vi "VIH ProjFile - Control Rules Array - Read.vi"(8 "error in":errorcluster, 10 "Property Name":string, 11 "XML Parent Item":refnum<k20>) -> (0 "error out":errorcluster, 1 "Control Rules":T1[](array[typedef]), 2 "Property found":bool, 3 "dup XML Parent Item":refnum<k20>)   [LabVIEW 2014]
doc: "::: VI Helpeks :::\nCopyright (c) 2000-2026 Konstantin Shifershteyn. All rights reserved."
uses:
  _VIH HelpGen.llb/VIH HelpGen Typedef - Cluster - Control Rule.ctl
  _VIH HelpGen.llb/VIH HelpGen Typedef - Enum - Description Mode.ctl
  _VIH HelpGen.llb/VIH HelpGen Typedef - Enum - Default,Enable,Disable.ctl
  _VIH HelpGen.llb/VIH HelpGen Typedef - Cluster - Enum Value Info.ctl
  <vilib>/xml/Close Reference(Node).vi
  <vilib>/xml/NI_XML.lvlib
panel:
  in  "Control Rule (data)":T1
  # "VI Helpeks\nCopyright (c) 2012-2026 Konstantin Shifershteyn"
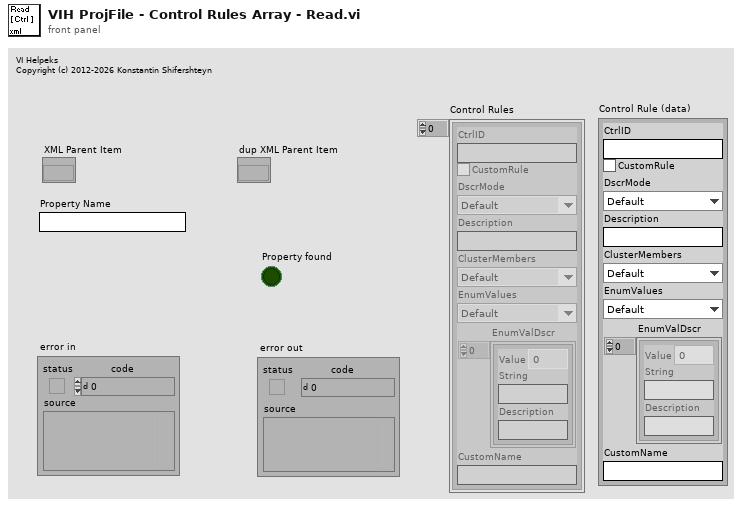
[diagram p1: front panel]
types:
  T1 = typedef "VIH HelpGen Typedef - Cluster - Control Rule.ctl" = cluster{"CtrlID":string, "CustomRule":bool, "DscrMode":T2, "Description":string, "ClusterMembers":T3, "EnumValues":T3, "EnumValDscr":T4[], "CustomName":string}
  T2 = typedef "VIH HelpGen Typedef - Enum - Description Mode.ctl" = enum16{"Default", "Description", "Description1", "Description2", "Custom", "None"}
  T3 = typedef "VIH HelpGen Typedef - Enum - Default,Enable,Disable.ctl" = enum16{"Default", "Enable", "Disable"}
  T4 = typedef "VIH HelpGen Typedef - Cluster - Enum Value Info.ctl" = cluster{"Value":ext, "String":string, "Description":string}
  T5 = typedef "KS HelpGen Typedef - Cluster - Control Rule.ctl" = cluster{"CtrlID":string, "CustomRule":bool, "DscrMode":T6, "Description":string, "ClusterMembers":T7, "EnumValues":T7, "EnumValDscr":T8[], "CustomName":string}
  T6 = typedef "KS HelpGen Typedef - Enum - Description Mode.ctl" = enum16{"Default", "Description", "Description1", "Description2", "Custom", "None"}
  T7 = typedef "KS HelpGen Typedef - Enum - Default,Enable,Disable.ctl" = enum16{"Default", "Enable", "Disable"}
  T8 = typedef "KS HelpGen Typedef - Cluster - Enum Value Info.ctl" = cluster{"Value":ext, "String":string, "Description":string}
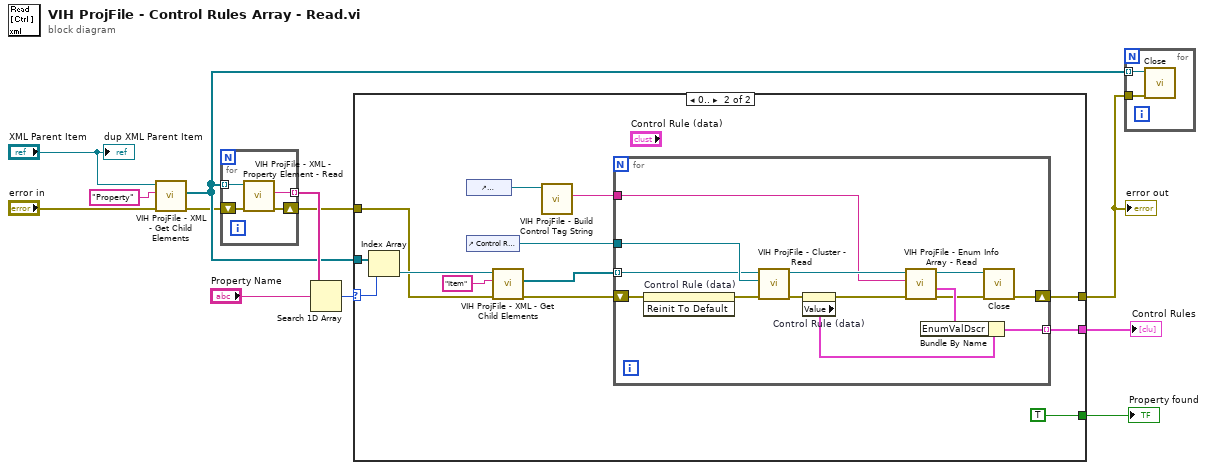
[diagram p0: block diagram]
diagram:
  n1 = call "VIH ProjFile - XML - Get Child Elements.vi"("error in"="error in", "Tag Name"="Property", "XML Parent Item"="XML Parent Item") -> ("error out"=w4:errorcluster, "Array of Elements"=w6:refnum<k20>[])  [unwired: 6 in, 1 out]
  n2 = for {
    tunnel: w6 -> [w16] mode=indexing
    shift-right: [w14] -> w10
    shift-left: w4 -> [w15]
    tunnel: [w13] -> w12 mode=indexing
    n3 = call "VIH ProjFile - XML - Property Element - Read.vi"("error in"=w15, "XML Node"=w16) -> ("error out"=w14:errorcluster, "Property Name"=w13:string)  [unwired: 6 in, 2 out]
  }
  n4 = Search 1D Array(1D array=w12, element="Property Name") -> (index of element=w11:i32)  [unwired: 1 in]
  n5 = case shown="0.." w11 {
    selector: w11 -> [_ w29]
    tunnel: [w17 w28] -> w8
    tunnel: w10 -> [w17 w22]
    tunnel: w6 -> [_ w30]
    tunnel: [_ w27] -> w9
    tunnel: [_ TRUE] -> w1
    frame ..-1 {
    }
    frame 0.. {
      n6 = Index Array(array=w30, index=w29) -> (element=w23:refnum<k20>)
      n7 = control-ref of="EnumValDscr"() -> (w26:refnum<vi>)
      n8 = control-ref of="Control Rule (data)"() -> (w25:refnum<vi>)
      n9 = call "VIH ProjFile - XML - Get Child Elements.vi"("error in"=w22, "Tag Name"="Item", "XML Parent Item"=w23) -> ("error out"=w20:errorcluster, "Array of Elements"=w21:refnum<k20>[])  [unwired: 6 in, 1 out]
      n10 = call "VIH ProjFile - Build Control Tag String.vi"("Ctl Refnum"=w26) -> ("Control Tag"=w24:string)  [unwired: 6 in, 4 out]
      n11 = for {
        tunnel: w21 -> [w31] mode=indexing
        shift-right: [w32] -> w28
        shift-left: w20 -> [w44]
        tunnel: [w35] -> w27 mode=indexing
        tunnel: w25 -> [w39]
        tunnel: w24 -> [w38]
        n12 = invoke on="Control Rule (data)" class="Clust (strict)" method="Reinit To Default"(error in=w44) -> (error out=w43:errorcluster)  [unwired: 2 in, 2 out]
        n13 = call "VIH ProjFile - Cluster - Read.vi"("error in"=w43, "Ctl Refnum"=w39, "XML Parent Item"=w31) -> ("error out"=w42:errorcluster, "dup XML Parent Item"=w40:refnum<k20>)  [unwired: 7 in]
        n14 = property on="Control Rule (data)" class="Clust (strict)"(error in=w42) -> (error out=w41:errorcluster, "Value"=w37:T5)  [unwired: 1 in, 1 out]
        n15 = call "VIH ProjFile - Enum Info Array - Read.vi"("error in"=w41, "Property Name"=w38, "XML Parent Item"=w40) -> ("error out"=w33:errorcluster, "EnumValDscr"=w36:T4[], "dup XML Parent Item"=w34:refnum<k20>)  [unwired: 5 in, 1 out]
        n16 = Bundle By Name(cluster=w37, "EnumValDscr"=w36) -> (w35:T5)
        n17 = call-poly <vilib>:"Close.vi"("error in (no error)"=w33, "node"=w34) -> ("error out"=w32:errorcluster)  [unwired: 7 in]
      }
    }
  }
  "error out" <- w8
  "Control Rules" <- w9
  "Property found" <- w1
  n18 = for {
    tunnel: w6 -> [w46] mode=indexing
    tunnel: w8 -> [w45]
    n19 = call-poly <vilib>:"Close.vi"("error in (no error)"=w45, "node"=w46) -> ()  [unwired: 7 in, 1 out]
  }
  "dup XML Parent Item" <- "XML Parent Item"
